vi "Circular Buffer (multiple).vi"(6 "History Length [1024]":i32=1024, 7 "reset":bool, 8 "error in":errorcluster, 11 "XY-data":cluster{"X-array":dbl[], "Y-array":dbl[]}[](array[cluster]) {"Y-array" format="%.2p"; "X-array" format="%.2p"}) -> (0 "error out":errorcluster, 3 "XY-data out":cluster{"X-array":dbl[], "Y-array":dbl[]}[](array[cluster]) {"Y-array" format="%.2p"; "X-array" format="%.2p"})   [LabVIEW 2019, in "xy_utilities.lvlib"]
doc: "Circular Buffer with controllable reset and history length."
uses:
  xy_utilities.lvlib
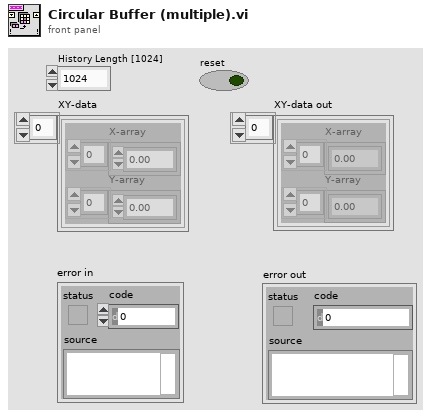
[diagram p1: front panel]
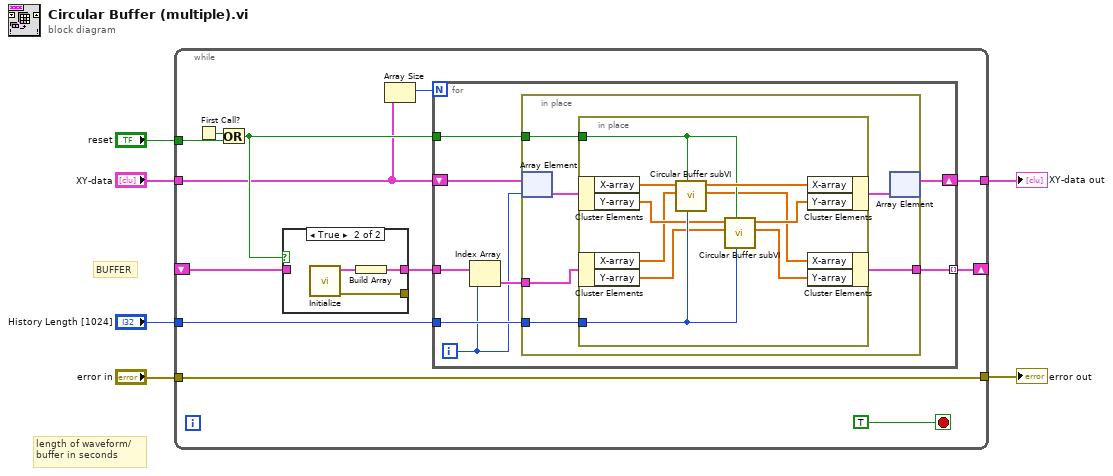
[diagram p0: block diagram]
diagram:
  # "BUFFER"
  # "length of waveform/\nbuffer in seconds"
  n1 = while {
    tunnel: "XY-data" -> [w7]
    tunnel: [w18] -> w3
    tunnel: "error in" -> [w18]
    tunnel: "reset" -> [w16]
    shift-right: [w13] -> _
    shift-left: _ -> [w11]
    tunnel: "History Length [1024]" -> [w14]
    tunnel: [w9] -> w1
    stop <- TRUE stop-if-true
    n2 = First Call?() -> (First Call?: T/F=w17:bool)
    n3 = Or(x=w17, y=w16) -> (x .or. y?=w10:bool)
    n4 = case shown="True" w10 {
      tunnel: w11 -> [w43 _]
      tunnel: [w43 w46] -> w12
      tunnel: [_ w44] -> _
      frame False {
      }
      frame True {
        n5 = call "Initialize.vi"() -> ("error out"=w44:errorcluster, "XY-data out"=w45:cluster{"X-array":dbl[], "Y-array":dbl[]})  [unwired: 10 in]
        n6 = Build Array(w45) -> (w46:cluster{"X-array":dbl[], "Y-array":dbl[]}[])
      }
    }
    n7 = Array Size(array=w7) -> (size(s)=w8:i32)
    n8 = for {
      N: w8 -> [_]
      tunnel: w14 -> [w26]
      tunnel: [w25] -> w13 mode=indexing
      tunnel: w12 -> [w22]
      tunnel: w10 -> [w24]
      shift-right: [w19] -> w9
      shift-left: w7 -> [w20]
      i -> [w21]
      n9 = Index Array(array=w22, index=w21) -> (element=w23:cluster{"X-array":dbl[], "Y-array":dbl[]})
      n10 = in-place {
        in-place-border: w26 -> [w32]
        in-place-border: [w31] -> w25
        in-place-border: w24 -> [w30]
        in-place-border: w23 -> [w29]
        n11 = in-place-array #1(w20, w21) -> (w28:cluster{"X-array":dbl[], "Y-array":dbl[]})
        n12 = in-place {
          in-place-border: w32 -> [w39]
          in-place-border: w30 -> [w40]
          n13 = in-place-cluster #2(w28) -> ("X-array"=w42:dbl[], "Y-array"=w37:dbl[])
          n14 = in-place-cluster #3(w29) -> ("X-array"=w36:dbl[], "Y-array"=w33:dbl[])
          n15 = call "Circular Buffer subVI.vi"("History Length [1024]"=w39, "Reset"=w40, "Buffer in"=w36, "Array in"=w42) -> ("Buffer out"=w34:dbl[], "Array out"=w41:dbl[])  [unwired: 6 in]
          n16 = call "Circular Buffer subVI.vi"("History Length [1024]"=w39, "Reset"=w40, "Buffer in"=w33, "Array in"=w37) -> ("Buffer out"=w35:dbl[], "Array out"=w38:dbl[])  [unwired: 6 in]
          n17 = in-place-cluster #2("X-array"=w41, "Y-array"=w38) -> (w27:cluster{"X-array":dbl[], "Y-array":dbl[]})
          n18 = in-place-cluster #3("X-array"=w34, "Y-array"=w35) -> (w31:cluster{"X-array":dbl[], "Y-array":dbl[]})
        }
        n19 = in-place-array #1(w27) -> (w19:cluster{"X-array":dbl[], "Y-array":dbl[]}[])  [unwired: 1 out]
      }
    }
  }
  "XY-data out" <- w1
  "error out" <- w3
